vi "LTE Handover.vi"(8 "error in (no error)":errorcluster caption="에러 입력(에러 없음)", 10 "LTE Call Handover Param":T1, 11 "Instrument Manager 입력":refnum<class "Instrument Manager.lvclass">) -> (0 "error out":errorcluster caption="에러 출력", 3 "Instrument Manager 출력":refnum<class "Instrument Manager.lvclass">)   [LabVIEW 2023, in "Instrument Manager.lvclass"]
uses:
  Instrument Manager.lvclass
  Type Definition/LTE Handover Param.ctl
  Module/ANRITSU Call Box/Type Definition/LTE Supported BandWidth.ctl
  75bd0187-fce6-41d7-bcb2-136bfaed1742.vi
  3ebe1be7-8bef-441d-a48b-cbbd9a1791ae.vi
  0d744e8d-db27-43c0-a0ed-b670d8860612.vi
  d5a6f7d3-30a6-4594-a940-10cc340811d9.vi
  59f82ec5-402a-4d8f-8cf3-640fd673fef9.vi
  Instrument Manager.lvclass/Instrument Manager.ctl
  Module/ANRITSU Call Box/ANRITSU Call Box.lvlib
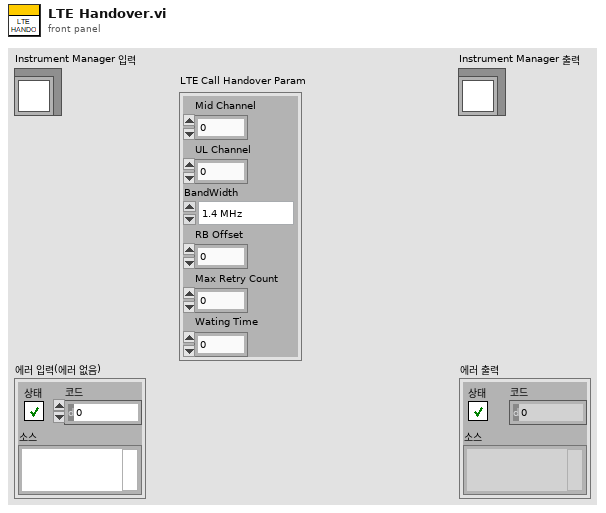
[diagram p1: front panel]
types:
  T1 = typedef "LTE Handover Param.ctl" = cluster{"Mid Channel":i32, "UL Channel":i32, "BandWidth":T2, "RB Offset":i32, "Max Retry Count":i32, "Wating Time":i32}
  T2 = typedef "ANRITSU Call Box.lvlib/LTE Supported BandWidth.ctl" = enum16{"1.4 MHz", "3 MHz", "5 MHz", "10 MHz", "15 MHz", "20 MHz"}
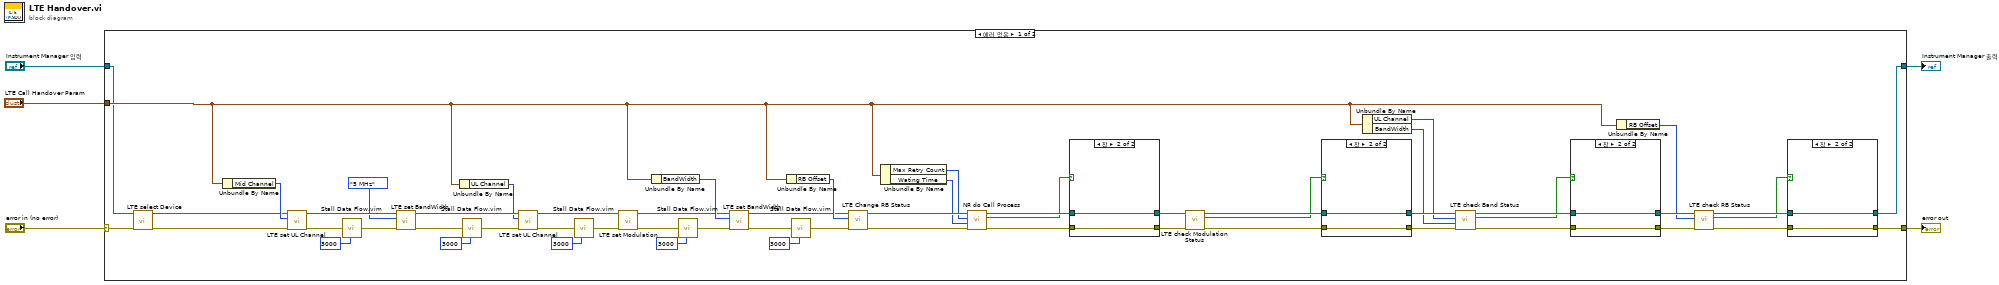
[diagram p0: block diagram]
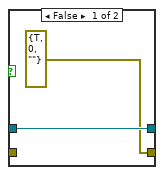
[diagram p2: hidden frame]
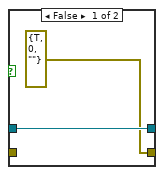
[diagram p3: hidden frame]
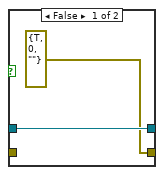
[diagram p4: hidden frame]
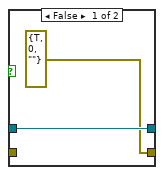
[diagram p5: hidden frame]
diagram:
  n1 = case shown="에러 없음" "error in (no error)" {
    selector: "error in (no error)" -> [w23 w80]
    tunnel: [w26 w80] -> w4
    tunnel: [w25 w79] -> w2
    tunnel: "Instrument Manager 입력" -> [w22 w79]
    tunnel: "LTE Call Handover Param" -> [w31 _]
    frame No Error {
      n2 = call "LTE select Device.vi"("error in (no error)"=w23, "Instrument Manager 입력"=w22) -> ("error out"=w24:errorcluster, "Instrument Manager 출력"=w21:refnum<class "Instrument Manager.lvclass">)  [unwired: 8 in]
      n3 = Unbundle By Name(w31) -> ("Mid Channel"=w62:i32)
      n4 = call "LTE set UL Channel.vi"("error in (no error)"=w24, "UL Channel"=w62, "Instrument Manager 입력"=w21) -> ("error out"=w19:errorcluster, "Instrument Manager 출력"=w61:refnum<class "Instrument Manager.lvclass">)  [unwired: 7 in]
      n5 = call "Stall Data Flow.vim"("value in"=w19, "milliseconds to wait"=u32 3000 ("millisecond timer value")) -> ("value out"=w18:errorcluster)  [unwired: 1 out]
      n6 = call "LTE set BandWidth.vi"("error in (no error)"=w18, "BandWidth"=LTE_Supported_BandWidth."5 MHz", "Instrument Manager 입력"=w61) -> ("error out"=w13:errorcluster, "Instrument Manager 출력"=w59:refnum<class "Instrument Manager.lvclass">)  [unwired: 7 in]
      n7 = Unbundle By Name(w31) -> ("UL Channel"=w58:i32)
      n8 = call "Stall Data Flow.vim"("value in"=w13, "milliseconds to wait"=u32 3000 ("millisecond timer value")) -> ("value out"=w12:errorcluster)  [unwired: 1 out]
      n9 = call "LTE set UL Channel.vi"("error in (no error)"=w12, "UL Channel"=w58, "Instrument Manager 입력"=w59) -> ("error out"=w11:errorcluster, "Instrument Manager 출력"=w57:refnum<class "Instrument Manager.lvclass">)  [unwired: 7 in]
      n10 = call "Stall Data Flow.vim"("value in"=w11, "milliseconds to wait"=u32 3000 ("millisecond timer value")) -> ("value out"=w10:errorcluster)  [unwired: 1 out]
      n11 = call "LTE set Modulation.vi"("error in (no error)"=w10, "Instrument Manager 입력"=w57) -> ("error out"=w9:errorcluster, "Instrument Manager 출력"=w55:refnum<class "Instrument Manager.lvclass">)  [unwired: 8 in]
      n12 = Unbundle By Name(w31) -> ("BandWidth"=w56:T2)
      n13 = call "Stall Data Flow.vim"("value in"=w9, "milliseconds to wait"=u32 3000 ("millisecond timer value")) -> ("value out"=w8:errorcluster)  [unwired: 1 out]
      n14 = call "LTE set BandWidth.vi"("error in (no error)"=w8, "BandWidth"=w56, "Instrument Manager 입력"=w55) -> ("error out"=w7:errorcluster, "Instrument Manager 출력"=w53:refnum<class "Instrument Manager.lvclass">)  [unwired: 7 in]
      n15 = Unbundle By Name(w31) -> ("RB Offset"=w54:i32)
      n16 = call "Stall Data Flow.vim"("value in"=w7, "milliseconds to wait"=u32 3000 ("millisecond timer value")) -> ("value out"=w6:errorcluster)  [unwired: 1 out]
      n17 = call "LTE Change RB Status.vi"("error in (no error)"=w6, "RB Offset"=w54, "Instrument Manager 입력"=w53) -> ("error out"=w52:errorcluster, "Instrument Manager 출력"=w51:refnum<class "Instrument Manager.lvclass">)  [unwired: 7 in]
      n18 = Unbundle By Name(w31) -> ("Max Retry Count"=w49:i32, "Wating Time"=w50:i32)
      n19 = call "NR do Call Process.vi"("error in (no error)"=w52, "Waiting Time"=w50, "Max Retry Count"=w49, "Instrument Manager 입력"=w51) -> ("error out"=w48:errorcluster, "Connected?"=w46:bool, "Instrument Manager 출력"=w47:refnum<class "Instrument Manager.lvclass">)  [unwired: 5 in]
      n20 = case shown="참" w46 {
        tunnel: w47 -> [w76 w78]
        tunnel: [w76 w78] -> w44
        tunnel: [errorcluster {"status"=TRUE, "code"=0, "source"=""} ("error out") w77] -> w45
        tunnel: w48 -> [_ w77]
        frame False {
        }
        frame True {
        }
      }
      n21 = call "LTE check Modulation Status.vi"("error in (no error)"=w45, "Instrument Manager 입력"=w44) -> ("error out"=w43:errorcluster, "불리언"=w41:bool, "Instrument Manager 출력"=w42:refnum<class "Instrument Manager.lvclass">)  [unwired: 7 in]
      n22 = case shown="참" w41 {
        tunnel: w42 -> [w72 w74]
        tunnel: [w72 w74] -> w39
        tunnel: [errorcluster {"status"=TRUE, "code"=0, "source"=""} ("error out") w73] -> w40
        tunnel: w43 -> [_ w73]
        frame False {
        }
        frame True {
        }
      }
      n23 = Unbundle By Name(w31) -> ("UL Channel"=w37:i32, "BandWidth"=w38:T2)
      n24 = call "LTE check Band Status.vi"("error in (no error)"=w40, "BandWidth"=w38, "UL Channel"=w37, "Instrument Manager 입력"=w39) -> ("error out"=w36:errorcluster, "불리언"=w34:bool, "Instrument Manager 출력"=w35:refnum<class "Instrument Manager.lvclass">)  [unwired: 5 in]
      n25 = case shown="참" w34 {
        tunnel: w35 -> [w68 w70]
        tunnel: [w68 w70] -> w32
        tunnel: [errorcluster {"status"=TRUE, "code"=0, "source"=""} ("error out") w69] -> w33
        tunnel: w36 -> [_ w69]
        frame False {
        }
        frame True {
        }
      }
      n26 = Unbundle By Name(w31) -> ("RB Offset"=w30:i32)
      n27 = call "LTE check RB Status.vi"("error in (no error)"=w33, "RB Offset"=w30, "Instrument Manager 입력"=w32) -> ("error out"=w29:errorcluster, "불리언"=w27:bool, "Instrument Manager 출력"=w28:refnum<class "Instrument Manager.lvclass">)  [unwired: 6 in]
      n28 = case shown="참" w27 {
        tunnel: w28 -> [w64 w66]
        tunnel: [w64 w66] -> w25
        tunnel: [errorcluster {"status"=TRUE, "code"=0, "source"=""} ("error out") w65] -> w26
        tunnel: w29 -> [_ w65]
        frame False {
        }
        frame True {
        }
      }
    }
    frame Error {
    }
  }
  "error out" <- w4
  "Instrument Manager 출력" <- w2
